vi "Set TTTR End Mode.vi"(8 "error in (no error)":errorcluster caption="错误输入（无错误）", 10 "uEvents64":u64, 11 "nEndMode":i32) -> (0 "error out":errorcluster caption="错误输出", 3 "function return":i32)   [LabVIEW 2017, in "smncsftmt.lvlib"]
doc: "__declspec(dllexport) int SetTTTREndMode(int nEndMode, unsigned long long uEvents64);"
uses:
  smncsftmt.lvlib
  smncsftmt.dll
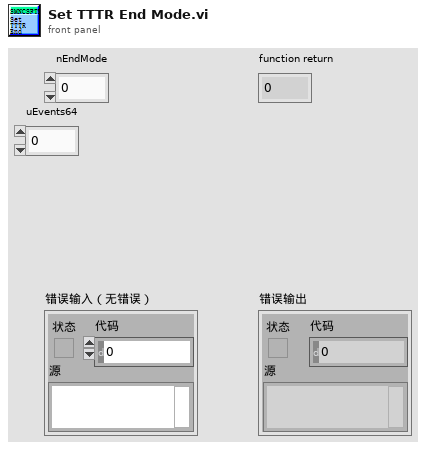
[diagram p1: front panel]
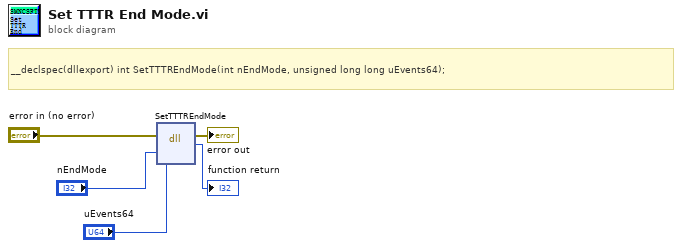
[diagram p0: block diagram]
diagram:
  # "__declspec(dllexport) int SetTTTREndMode(int nEndMode, unsigned long long uEvents64);"
  n1 = dll-call lib="PTH2oabs CUsersaDesktop\nLABVIEW范例National InstrumentsLabVIEW 2017user.lib\tsmncsftmtsmncsftmt.*" fn="SetTTTREndMode"(error in="error in (no error)", "nEndMode"="nEndMode", "uEvents64"="uEvents64") -> (error out=→"error out":errorcluster, "返回类型"=→"function return":i32)  [unwired: 4 in, 1 out]
